vi "Parse Sequence JSON.vi"(8 "error in":errorcluster, 11 "JSON string":string) -> (0 "error out":errorcluster, 3 "Sequence File":T1)   [LabVIEW 2026]
doc: "Parses a sequence JSON document into a Sequence File cluster with Unflatten From JSON; the JSON keys equal the typedef field labels. A JSON parse error is passed out unchanged. If the document parses but its steps array is empty, error 5001 \"sequence has no steps\" is returned. An incoming error skips the parse. AF-free."
uses:
  Typedefs/Sequence File.ctl
  Typedefs/Step Config.ctl
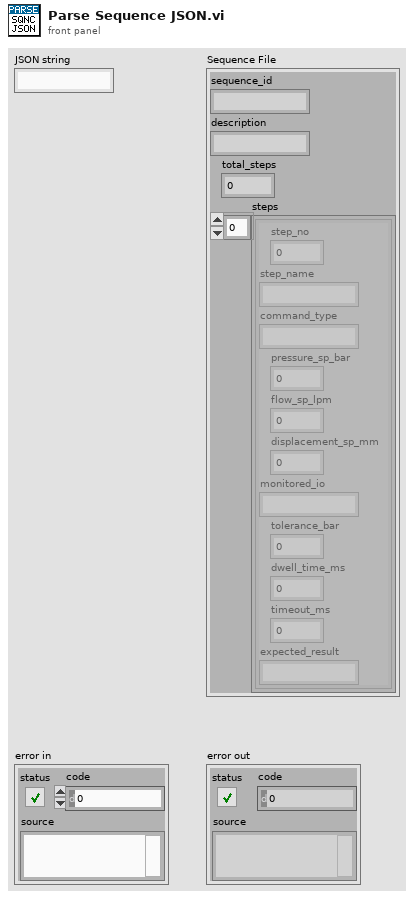
[diagram p1: front panel]
types:
  T1 = typedef "Sequence File.ctl" = cluster{"sequence_id":string, "description":string, "total_steps":i32, "steps":T2[]}
  T2 = typedef "Step Config.ctl" = cluster{"step_no":i32, "step_name":string, "command_type":string, "pressure_sp_bar":dbl, "flow_sp_lpm":dbl, "displacement_sp_mm":dbl, "monitored_io":string, "tolerance_bar":dbl, "dwell_time_ms":i32, "timeout_ms":i32, "expected_result":string}
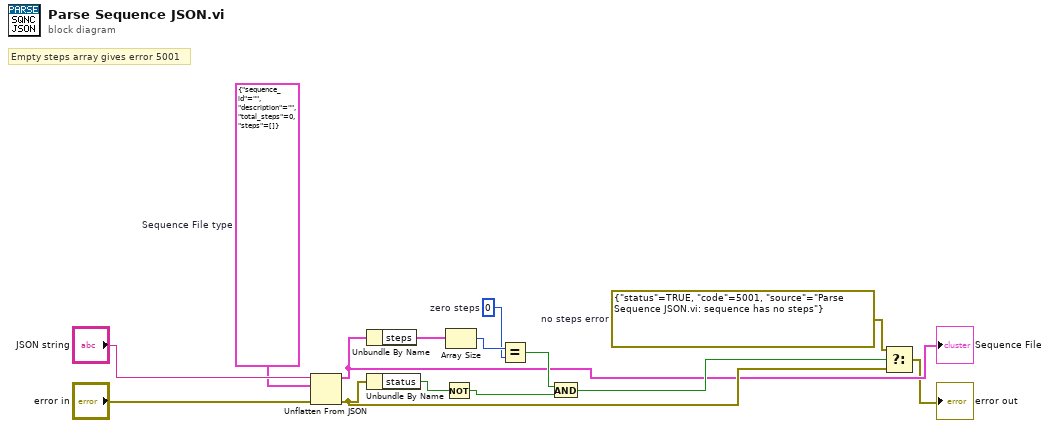
[diagram p0: block diagram]
diagram:
  w4 = errorcluster {"status"=TRUE, "code"=5001, "source"="Parse Sequence JSON.vi: sequence has no steps"}  # no steps error
  w9 = 0  # zero steps
  w13 = T1 {"sequence_id"="", "description"="", "total_steps"=0, "steps"=[]}  # Sequence File type
  # "Empty steps array gives error 5001"
  n1 = Unflatten From JSON(JSON string="JSON string", type and defaults=w13, error in (no error)="error in") -> (value=w2:T1, error out=w3:errorcluster)  [unwired: 4 in]
  "Sequence File" <- w2
  n2 = Unbundle By Name(w2) -> ("steps"=w11:T2[])
  n3 = Unbundle By Name(w3) -> ("status"=w8:bool)
  n4 = Not(x=w8) -> (.not. x?=w6:bool)
  n5 = Array Size(array=w11) -> (size(s)=w10:i32)
  n6 = Equal?(x=w10, y=w9) -> (x = y?=w7:bool)
  n7 = And(x=w7, y=w6) -> (x .and. y?=w5:bool)
  n8 = Select(t=w4, s=w5, f=w3) -> (s? t:f=→"error out":errorcluster)
